vi "Test_WS_Close.vi"() -> ()   [LabVIEW 2021]
doc: "C6 test: before_ws, TLS connect, WebSocket handshake, after_ws (2 filters), then holds the WebSocket open until Stop for curl checks. Closes TCP only; free the channel with curl DELETE /api/can/<ch>/ws until C7 exists."
uses:
  common/CANsub_Common.lvlib
  common/Typedefs/REST_Phase.ctl
  common/Typedefs/Bit_Timing.ctl
panel:
  out "closed by device":bool
  out "error out":errorcluster
  out "leftover bytes":i32
  out "headers":string
  out "nodelay":i32
  out "api version":string
  in  "stop":bool
  in  "bit timing":T1={"brp"=2, "seg1"=63, "seg2"=16, "sjw"=16, "data brp"=2, "data seg1"=15, "data seg2"=4, "data sjw"=4}
  in  "cert path":path=path "/home/lvuser/cansub_root_cert.crt"
  in  "channel":u8=2
  in  "host":string="192.168.0.49"
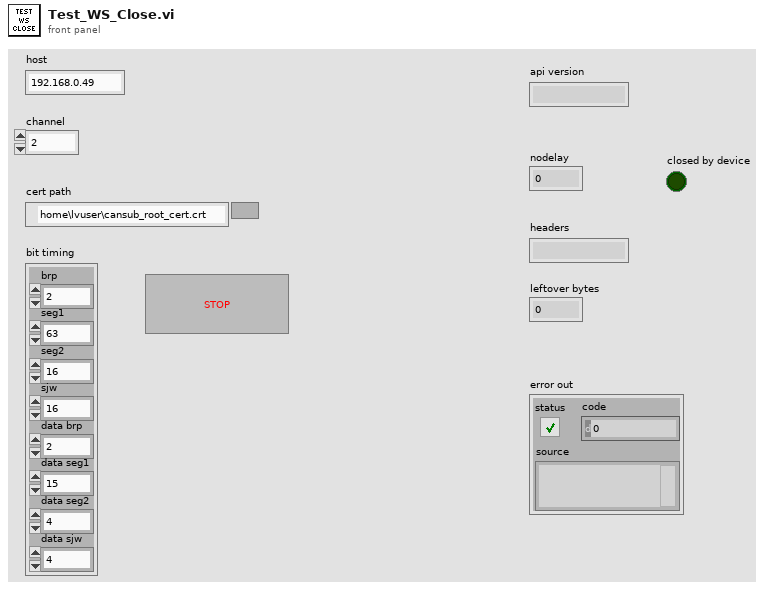
[diagram p1: front panel]
types:
  T1 = typedef "CANsub_Common.lvlib/Bit_Timing.ctl" = cluster{"brp":u16, "seg1":u16, "seg2":u16, "sjw":u16, "data brp":u16, "data seg1":u16, "data seg2":u16, "data sjw":u16}
  T2 = typedef "CANsub_Common.lvlib/REST_Phase.ctl" = enum16{"before_ws", "after_ws"}
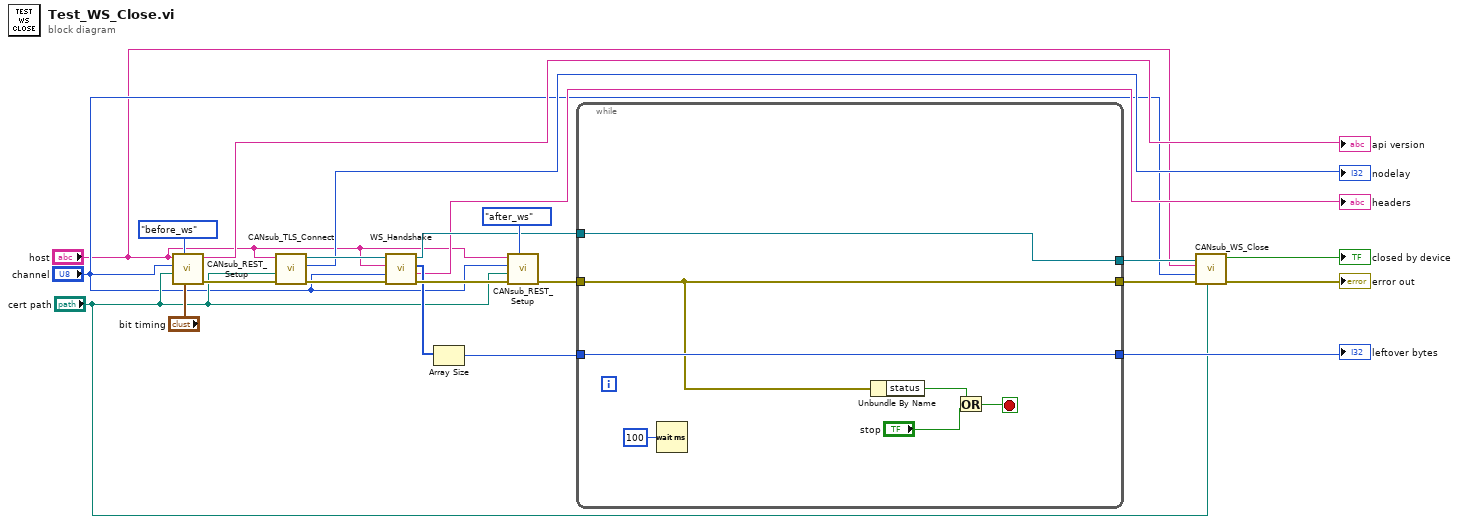
[diagram p0: block diagram]
diagram:
  n1 = call "CANsub_REST_Setup.vi"("bit timing"="bit timing", "phase"=REST_Phase."before_ws", "cert path"="cert path", "channel"="channel", "host"="host") -> ("error out"=w22:errorcluster, "api version"=→"api version":string)  [unwired: 5 in]
  n2 = call "CANsub_TLS_Connect.vi"("error in (no error)"=w22, "cert path"="cert path", "host"="host") -> ("error out"=w21:errorcluster, "nodelay"=→"nodelay":i32, "TLS connection"=w16:refnum<k5>)  [unwired: 6 in]
  n3 = call "WS_Handshake.vi"("error in (no error)"=w21, "channel"="channel", "host"="host", "TLS connection"=w16) -> ("error out"=w20:errorcluster, "headers"=→"headers":string, "leftover"=w15:u8[], "TLS connection out"=w11:refnum<k5>)  [unwired: 4 in]
  n4 = Array Size(array=w15) -> (size(s)=w13:i32)
  n5 = call "CANsub_REST_Setup.vi"("phase"=REST_Phase."after_ws", "error in (no error)"=w20, "cert path"="cert path", "channel"="channel", "host"="host") -> ("error out"=w19:errorcluster)  [unwired: 5 in, 1 out]
  n6 = while {
    tunnel: w19 -> [w27]
    tunnel: [w29] -> w14
    tunnel: w13 -> [w29]
    tunnel: [w27] -> w6
    tunnel: [w23] -> w7
    tunnel: w11 -> [w23]
    stop <- w24 stop-if-true
    n7 = Wait (ms)(milliseconds to wait=u32 100) -> ()  [unwired: 1 out]
    n8 = Unbundle By Name(w27) -> ("status"=w26:bool)
    n9 = Or(x=w26, y="stop") -> (x .or. y?=w24:bool)
  }
  "leftover bytes" <- w14
  n10 = call "CANsub_WS_Close.vi"("cert path"="cert path", "error in (no error)"=w6, "channel"="channel", "host"="host", "TLS Connection"=w7) -> ("error out"=→"error out":errorcluster, "closed by device"=→"closed by device":bool)  [unwired: 5 in]
